vi "十字路口仿真V1.vi"() -> ()   [LabVIEW 2014]
panel:
  out "loop_count":dbl
  in  "停止":bool
  in  "step_ms":dbl
  out "slice_name":string
  out "cycle_no":dbl
  out "remain_s":dbl
  out "t_s":dbl
  out "EW_LT_G":bool
  out "EW_TH_G":bool
  out "NS_LT_G":bool
  out "NS_TH_G":bool
  out "EW_LT_Y":bool
  out "EW_TH_Y":bool
  out "NS_LT_Y":bool
  out "NS_TH_Y":bool
  out "EW_LT_R":bool
  out "EW_TH_R":bool
  out "NS_LT_R":bool
  out "NS_TH_R":bool
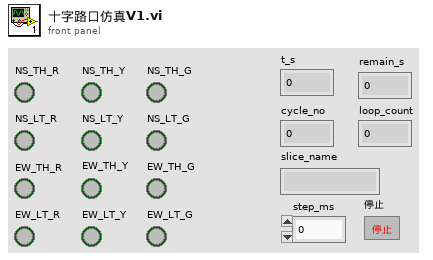
[diagram p1: front panel]
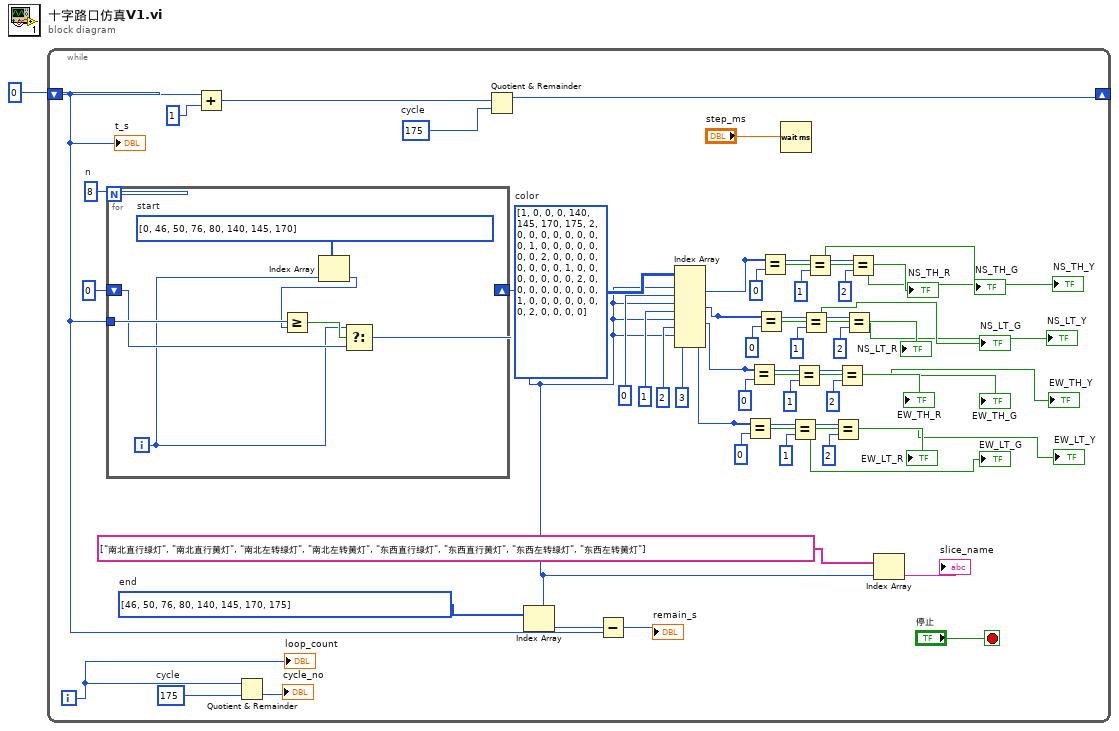
[diagram p0: block diagram]
diagram:
  n1 = while {
    shift-right: [w48] -> _
    shift-left: 0 -> [w9]
    i -> [w3]
    stop <- "停止" stop-if-true
    w5 = 175  # cycle
    w12 = i32[] [46, 50, 76, 80, 140, 145, 170, 175]  # end
    w33 = i32[][] [[1, 0, 0, 0, 140, 145, 170, 175], [2, 0, 0, 0, 0, 0, 0, 0], [0, 1, 0, 0, 0, 0, 0, 0], [0, 2, 0, 0, 0, 0, 0, 0], [0, 0, 1, 0, 0, 0, 0, 0], [0, 0, 2, 0, 0, 0, 0, 0], [0, 0, 0, 1, 0, 0, 0, 0], [0, 0, 0, 2, 0, 0, 0, 0]]  # color
    w47 = 8  # n
    w49 = 175  # cycle
    n2 = for {
      N: w47 -> [_]
      shift-right: [w55] -> w8
      shift-left: 0 -> [w56]
      tunnel: w9 -> [w58]
      i -> [w53]
      w59 = i32[] [0, 46, 50, 76, 80, 140, 145, 170]  # start
      n3 = Index Array(array=w59, index=w53) -> (element=w54:i32)
      n4 = Greater Or Equal?(x=w58, y=w54) -> (x >= y?=w57:bool)
      n5 = Select(t=w53, s=w57, f=w56) -> (s? t:f=w55:i32)
    }
    n6 = Add(x=w9, y=1) -> (x+y=w50:i32)
    n7 = Quotient & Remainder(x=w3, y=w5) -> (floor(x/y)=→"cycle_no":i32)  [unwired: 1 out]
    n8 = Quotient & Remainder(x=w50, y=w49) -> (x-y*floor(x/y)=w48:i32)  [unwired: 1 out]
    n9 = Index Array(array=w12, index=w8) -> (element=w11:i32)
    n10 = Subtract(x=w11, y=w9) -> (x-y=→"remain_s":i32)
    n11 = Index Array(array=w33, index (row) #1=w8, index (col) #1=0, index (row) #2=w8, index (col) #2=1, index (row) #3=w8, index (col) #3=2, index (row) #4=w8, index (col) #4=3) -> (element #1=w28:i32, element #2=w27:i32, element #3=w26:i32, element #4=w25:i32)
    n12 = Equal?(x=w25, y=0) -> (x = y?=→"EW_LT_R":bool)
    n13 = Equal?(x=w26, y=0) -> (x = y?=→"EW_TH_R":bool)
    n14 = Equal?(x=w27, y=0) -> (x = y?=→"NS_LT_R":bool)
    n15 = Equal?(x=w28, y=0) -> (x = y?=→"NS_TH_R":bool)
    n16 = Wait (ms)(milliseconds to wait="step_ms") -> ()  [unwired: 1 out]
    n17 = Equal?(x=w25, y=1) -> (x = y?=→"EW_LT_G":bool)
    n18 = Equal?(x=w26, y=1) -> (x = y?=→"EW_TH_G":bool)
    n19 = Equal?(x=w27, y=1) -> (x = y?=→"NS_LT_G":bool)
    n20 = Equal?(x=w28, y=1) -> (x = y?=→"NS_TH_G":bool)
    n21 = Equal?(x=w25, y=2) -> (x = y?=→"EW_LT_Y":bool)
    n22 = Equal?(x=w26, y=2) -> (x = y?=→"EW_TH_Y":bool)
    n23 = Equal?(x=w27, y=2) -> (x = y?=→"NS_LT_Y":bool)
    n24 = Equal?(x=w28, y=2) -> (x = y?=→"NS_TH_Y":bool)
    n25 = Index Array(array=string[] ["南北直行绿灯", "南北直行黄灯", "南北左转绿灯", "南北左转黄灯", "东西直行绿灯", "东西直行黄灯", "东西左转绿灯", "东西左转黄灯"], index=w8) -> (element=→"slice_name":string)
    "t_s" <- w9
    "loop_count" <- w3
  }
